vi "Excess-64-Byte-Array-to-Real.vi"(4 "Byte array (4 or 8 bytes)":u8[](array[numeric]) format="%08x") -> (1 "Real Number":dbl)   [LabVIEW 2019]
panel:
  # "42 5A 00 00 00 00 00 00"
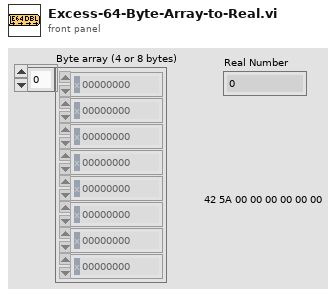
[diagram p1: front panel]
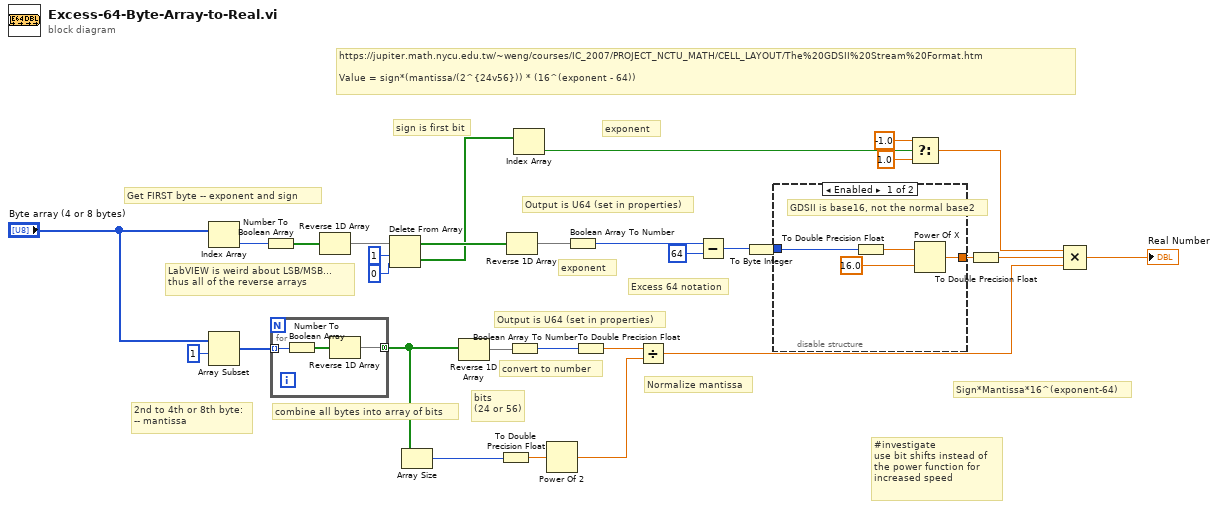
[diagram p0: block diagram]
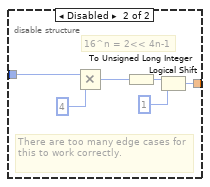
[diagram p2: hidden frame]
diagram:
  # "#investigate\nuse bit shifts instead of the power function for increased speed"
  # "exponent"
  # "bits\n(24 or 56)"
  # "Output is U64 (set in properties)"
  # "https://jupiter.math.nycu.edu.tw/~weng/courses/IC_2007/PROJECT_NCTU_MATH/CELL_LAYOUT/The%20GDSII%20Stream%20Format.htm\n\nValue = sign*(mantissa/(2^{24v56})) * (16^(exponent - 64))"
  # "combine all bytes into array of bits"
  # "LabVIEW is weird about LSB/MSB... thus all of the reverse arrays"
  # "2nd to 4th or 8th byte:\n-- mantissa"
  # "Sign*Mantissa*16^(exponent-64)"
  # "Excess 64 notation"
  # "convert to number"
  # "Normalize mantissa"
  # "exponent"
  # "sign is first bit"
  # "Get FIRST byte -- exponent and sign"
  # "Output is U64 (set in properties)"
  n1 = Index Array(array="Byte array (4 or 8 bytes)") -> (element=w12:u8)  [unwired: 1 in]
  n2 = Array Subset(array="Byte array (4 or 8 bytes)", index=1) -> (w19:u8[])  [unwired: 1 in]
  n3 = Number To Boolean Array(number=w12) -> (Boolean array=w18:bool[])
  n4 = for {
    tunnel: w19 -> [w32] mode=indexing
    tunnel: [w30] -> w13 mode=concatenating
    n5 = Number To Boolean Array(number=w32) -> (Boolean array=w31:bool[])
    n6 = Reverse 1D Array(array=w31) -> (reversed array=w30:bool[])
  }
  n7 = Reverse 1D Array(array=w18) -> (reversed array=w16:bool[])
  n8 = Delete From Array(array=w16, length=1, index=0) -> (deleted portion=w15:bool[], array with subset deleted=w22:bool[])
  n9 = Array Size(array=w13) -> (size(s)=w14:i32)
  n10 = Reverse 1D Array(array=w13) -> (reversed array=w24:bool[])
  n11 = To Double Precision Float(number=w14) -> (double precision float=w4:dbl)
  n12 = Reverse 1D Array(array=w22) -> (reversed array=w29:bool[])
  n13 = Boolean Array To Number(Boolean array=w24) -> (number=w25:u64)
  n14 = Index Array(array=w15) -> (element=w9:bool)  [unwired: 1 in]
  n15 = Power Of 2(x=w4) -> (2^x=w20:dbl)
  n16 = Boolean Array To Number(Boolean array=w29) -> (number=w26:u64)
  n17 = To Double Precision Float(number=w25) -> (double precision float=w3:dbl)
  n18 = Divide(x=w3, y=w20) -> (x/y=w10:dbl)
  n19 = Subtract(x=w26, y=u64 64) -> (x-y=w28:u64)
  n20 = disable-structure shown="Enabled" {
    disable-tunnel: w28 -> [w36 w39]
    disable-tunnel: [w33 w42] -> w2
    frame Enabled {
      # "GDSII is base16, not the normal base2"
      n21 = To Byte Integer(number=w36) -> (8bit integer=w34:i8)
      n22 = To Double Precision Float(number=w34) -> (double precision float=w37:dbl)
      n23 = Power Of X(1:16.0 ("x"), 2:w37) -> (0:w33:dbl)
    }
    frame Disabled {
      # "There are too many edge cases for this to work correctly."
      # "16^n = 2<< 4n-1"
      n24 = Multiply(x=w39, y=u64 4) -> (x*y=w38:u64)
      n25 = To Unsigned Long Integer(number=w38) -> (unsigned 32bit integer=w41:u32)
      n26 = Logical Shift(y=w41, x=u32 1) -> (x << y=w42:u32)
    }
  }
  n27 = Select(t=-1.0, s=w9, f=1.0) -> (s? t:f=w6:dbl)
  n28 = To Double Precision Float(number=w2) -> (double precision float=w1:dbl)
  n29 = Compound Arithmetic op=MULTIPLY(w6, w1, w10) -> (→"Real Number":dbl)
